vi "OnCFXMessageReceived.vi"(4 "CFX_message":refnum<vi>, 5 "事件数据":T1, 6 "控件引用":refnum<k24>, 7 "事件通用数据":cluster{"事件源":i32, "事件类型":u32, "时间标识":u32}) -> ()   [LabVIEW 2025]
uses:
  CFX_dll/CFX.dll
  SubVI/table/1 model/a log/_myType runlog cmd.ctl
panel:
  out "error out":errorcluster caption="错误输出"
  in  "error in":errorcluster caption="错误输入"
  out "SupportedTopicQueryType":i32(ring) items=["All", "Any", "Ignore"]
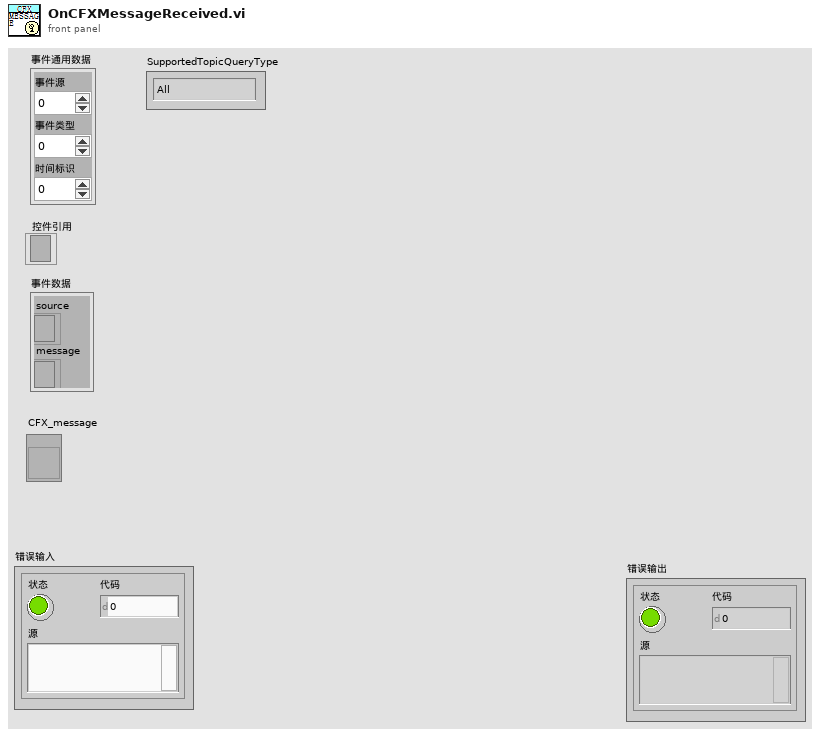
[diagram p1: front panel]
types:
  T1 = cluster{"source":refnum<k24>, "message":refnum<k24>}
  T2 = typedef "_myType runlog cmd.ctl" = enum16{"init", "push (-1: error)", "push (0: user)", "push (1: logical)", "push (2: driver)", "push (3: lib-core)", "push (4: reserved)", "pop", "more?"}
  T3 = cluster{"Message_Name":string, "CFX_Handle":string, "Message_Content":string}
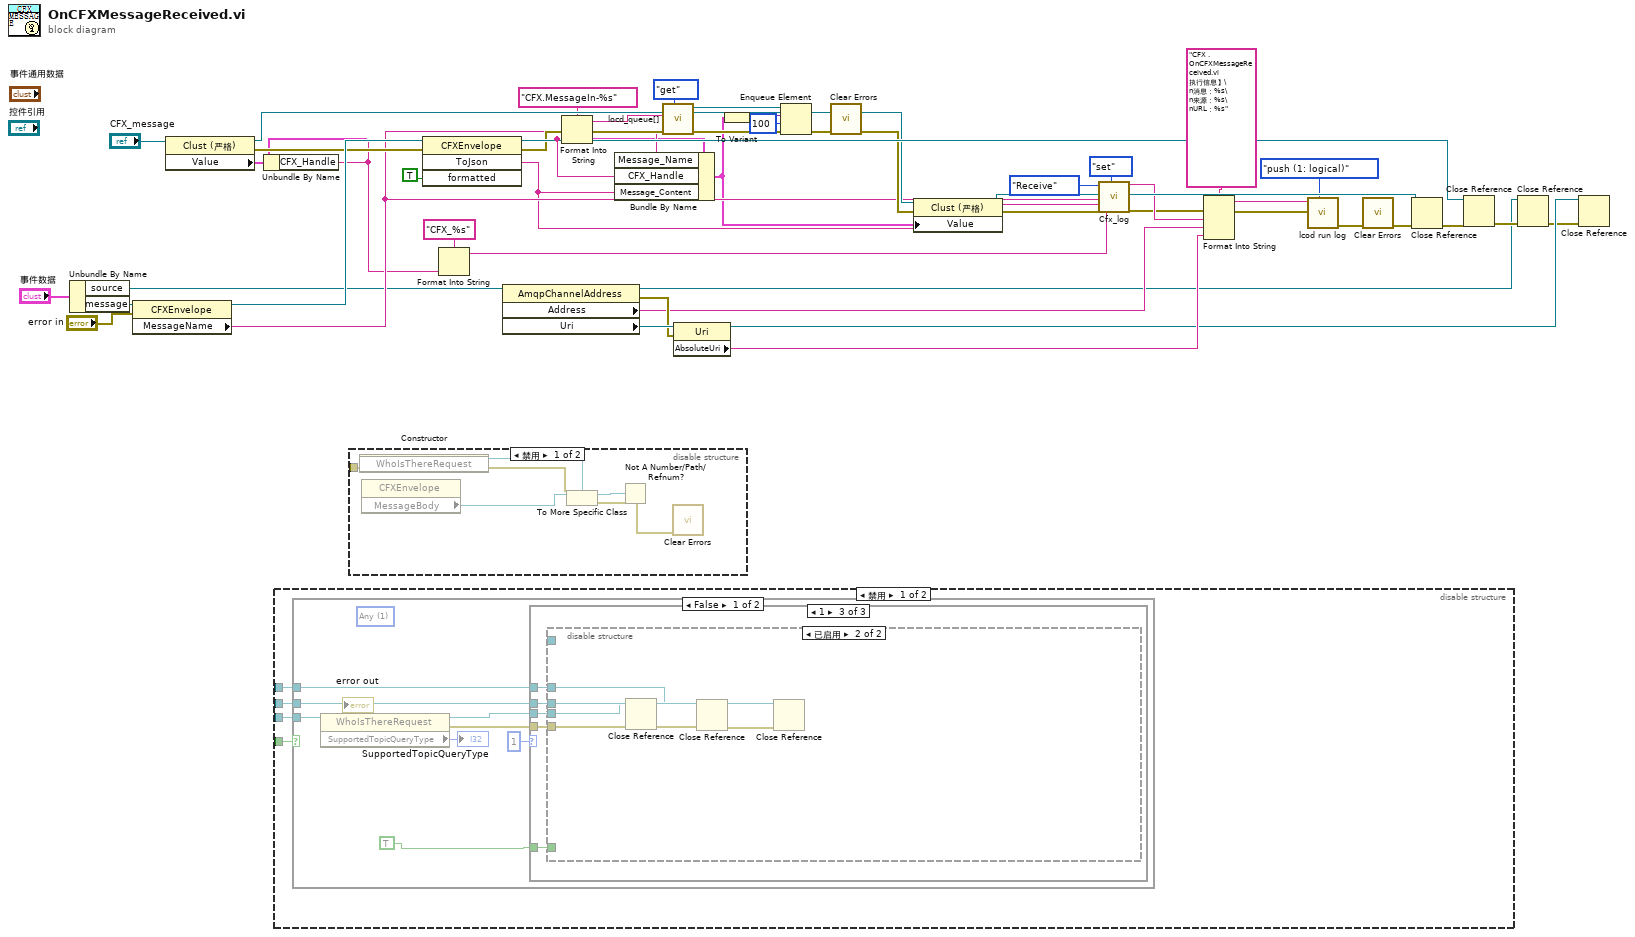
[diagram p0: block diagram]
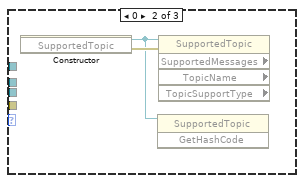
[diagram p4: hidden frame]
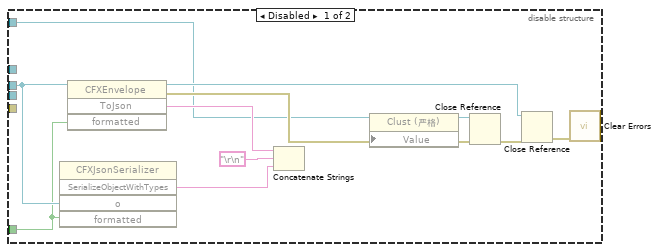
[diagram p5: hidden frame]
diagram:
  n1 = Unbundle By Name("事件数据") -> ("source"=w10:refnum<k24>, "message"=w48:refnum<k24>)
  n2 = property on="属性节点" class="CFXEnvelope"(reference=w48, error in="error in") -> (reference out=w45:refnum<k24>, "MessageName"=w25:string)  [unwired: 1 out]
  n3 = property class="Clust (严格)"(reference="CFX_message") -> (reference out=w34:refnum<vi>, error out=w30:errorcluster, "Value"=w1:T3)  [unwired: 1 in]
  n4 = Unbundle By Name(w1) -> ("CFX_Handle"=w24:string)
  n5 = disable-structure shown="禁用" {
    disable-tunnel: _ -> [w53 _]
    disable-tunnel: _ -> [w52 _]
    disable-tunnel: _ -> [w51 _]
    disable-tunnel: _ -> [w50 _]
    frame Disabled {
      n6 = case shown="False" w52 {
        tunnel: w51 -> [w61 _]
        tunnel: w50 -> [w56 _]
        tunnel: w53 -> [w60 _]
        frame False {
          (unwired) 1 items=["All", "Any", "Ignore"] ("SupportedTopicQueryType")
          n7 = property on="属性节点" class="WhoIsThereRequest"(reference=w60) -> (reference out=w55:refnum<k24>, error out=w57:errorcluster, "SupportedTopicQueryType"=→"SupportedTopicQueryType":i32)  [unwired: 1 in]
          n8 = case shown="1" 1 ("SupportedTopicQueryType") {
            tunnel: w61 -> [_ _ w68]
            tunnel: TRUE ("formatted") -> [_ _ w67]
            tunnel: w57 -> [_ _ w66]
            tunnel: w56 -> [_ _ w65]
            tunnel: w55 -> [_ _ w64]
            frame 99, Default {
            }
            frame 0 {
              n9 = constructor class="SupportedTopic"() -> (reference out=w62:refnum<k24>, error out=w63:errorcluster)  [unwired: 3 in, 1 out]
              n10 = invoke class="SupportedTopic" method="GetHashCode"(reference=w62) -> ()  [unwired: 2 in, 3 out]
              n11 = property on="属性节点" class="SupportedTopic" props=["SupportedMessages", "TopicName", "TopicSupportType"](reference=w62, error in=w63) -> ()  [unwired: 5 out]
            }
            frame 1 {
              n12 = disable-structure shown="已启用" {
                disable-tunnel: w68 -> [w73 w86]
                disable-tunnel: w67 -> [w72 _]
                disable-tunnel: _ -> [w71 _]
                disable-tunnel: w66 -> [_ w85]
                disable-tunnel: w65 -> [_ w83]
                disable-tunnel: w64 -> [_ w81]
                frame Disabled {
                  n13 = invoke on="调用节点" class="CFXJsonSerializer" method="SerializeObjectWithTypes"("o"=w73, "formatted"=w72) -> ("SerializeObjectWithTypes"=w74:string)  [unwired: 3 in, 4 out]
                  n14 = invoke on="调用节点" class="CFXEnvelope" method="ToJson"(reference=w73, "formatted"=w72) -> (reference out=w79:refnum<k24>, error out=w77:errorcluster, "ToJson"=w78:string)  [unwired: 2 in, 1 out]
                  n15 = Concatenate Strings(w78, "\r\n", w74) -> ()  [unwired: 1 out]
                  n16 = property class="Clust (严格)" props=["Value"](reference=w71, error in=w77) -> (reference out=w70:refnum<vi>, error out=w69:errorcluster)  [unwired: 1 in]
                  n17 = Close Reference(reference=w70, error in (no error)=w69) -> (error out=w80:errorcluster)
                  n18 = Close Reference(reference=w79, error in (no error)=w80) -> (error out=w76:errorcluster)
                  n19 = call <vilib>:"Clear Errors.vi"("error in (no error)"=w76) -> ()  [unwired: 5 in, 2 out]
                }
                frame Enabled {
                  n20 = Close Reference(reference=w81, error in (no error)=w85) -> (error out=w82:errorcluster)
                  n21 = Close Reference(reference=w86, error in (no error)=w82) -> (error out=w84:errorcluster)
                  n22 = Close Reference(reference=w83, error in (no error)=w84) -> ()  [unwired: 1 out]
                }
              }
            }
          }
        }
        frame True {
        }
      }
    }
    frame Enabled {
    }
  }
  n23 = disable-structure shown="禁用" {
    disable-tunnel: _ -> [w88 _]
    frame Disabled {
      n24 = constructor class="WhoIsThereRequest"(error in=w88) -> (reference out=w92:refnum<k24>, error out=w89:errorcluster)  [unwired: 2 in, 1 out]
      n25 = property on="属性节点" class="CFXEnvelope"() -> ("MessageBody"=w87:refnum<k24>)  [unwired: 2 in, 2 out]
      n26 = To More Specific Class(target class=w92, reference=w87, error in=w89) -> (specific class reference=w91:refnum<k24>, error out=w90:errorcluster)
      n27 = Not A Number/Path/Refnum?(number/path/refnum=w91) -> ()  [unwired: 1 out]
      n28 = call <vilib>:"Clear Errors.vi"("error in (no error)"=w90) -> ()  [unwired: 5 in, 2 out]
    }
    frame Enabled {
    }
  }
  n29 = invoke on="调用节点" class="CFXEnvelope" method="ToJson"(reference=w45, error in=w30, "formatted"=TRUE) -> (reference out=w47:refnum<k24>, error out=w29:errorcluster, "ToJson"=w23:string)  [unwired: 1 in, 1 out]
  n30 = Format Into String(format string="CFX_%s" ("log_path"), w24) -> (resulting string=w26:string)  [unwired: 2 in, 1 out]
  n31 = property class="AmqpChannelAddress"(reference=w10) -> (reference out=w4:refnum<k24>, error out=w8:errorcluster, "Address"=w7:string, "Uri"=w9:refnum<k24>)  [unwired: 1 in]
  n32 = Format Into String(format string="CFX.MessageIn-%s" ("格式字符串"), error in=w29, w24) -> (resulting string=w32:string, error out=w28:errorcluster)  [unwired: 1 in]
  n33 = Bundle By Name(cluster=w1, "Message_Name"=w25, "CFX_Handle"=w24, "Message_Content"=w23) -> (w22:T3)
  n34 = call "locd_queue[].vi"("cmd"=enum16{"init", "get", "set", "end"}."get", "error in"=w28, "queue_name"=w32) -> ("error out"=w38:errorcluster, "queue_out"=w40:refnum<queue>)  [unwired: 4 in, 3 out]
  n35 = property class="Uri"(reference=w9, error in=w8) -> (reference out=w3:refnum<k24>, "AbsoluteUri"=w6:string)  [unwired: 1 out]
  n36 = To Variant(anything=w22) -> (Variant=w39:variant)
  n37 = Enqueue Element(queue=w40, element=w39, timeout in ms (-1)=100 ("超时毫秒(-1)"), error in (no error)=w38) -> (error out=w36:errorcluster)  [unwired: 2 out]
  n38 = call <vilib>:"Clear Errors.vi"("error in (no error)"=w36) -> ("error out"=w31:errorcluster)  [unwired: 5 in, 1 out]
  n39 = property class="Clust (严格)"(reference=w34, error in=w31, "Value"=w22) -> (reference out=w42:refnum<vi>, error out=w12:errorcluster)
  n40 = call "Cfx_log.vi"("R/W"=enum16{"Send", "Receive"}."Receive" ("cmd"), "Message_Name"=w25, "Message_Content"=w23, "error in"=w12, "log_path"=w26, "cmd"=enum16{"init", "set", "save"}."set") -> ("Log_out"=w15:string, "error out"=w14:errorcluster)  [unwired: 12 in]
  n41 = Format Into String(format string="CFX .OnCFXMessageReceived.vi 执行信息】\n消息：%s\n来源：%s\nURL：%s", error in=w14, w15, w7, w6) -> (resulting string=w18:string, error out=w19:errorcluster)  [unwired: 1 in]
  n42 = call "lcod run log.vi"("cmd"=_myType_runlog_cmd."push (1: logical)", "Error In"=w19, "str in"=w18) -> ("Error Out"=w13:errorcluster)  [unwired: 6 in, 2 out]
  n43 = call <vilib>:"Clear Errors.vi"("error in (no error)"=w13) -> ("error out"=w11:errorcluster)  [unwired: 5 in, 1 out]
  n44 = Close Reference(reference=w42, error in (no error)=w11) -> (error out=w46:errorcluster)
  n45 = Close Reference(reference=w47, error in (no error)=w46) -> (error out=w5:errorcluster)
  n46 = Close Reference(reference=w4, error in (no error)=w5) -> (error out=w2:errorcluster)
  n47 = Close Reference(reference=w3, error in (no error)=w2) -> ()  [unwired: 1 out]
